vi "Open.vi"(8 "error in (no error)":errorcluster, 10 "App Refnum":refnum<vi>, 11 "LVUnit Test Case in":refnum<class "LVUnit Test Case.lvclass">) -> (0 "error out":errorcluster, 3 "LVUnit Test Case out":refnum<class "LVUnit Test Case.lvclass">)   [LabVIEW 2017, in "LVUnit Test Case.lvclass"]
doc: "Opens the document associated with the test case in the provided application context."
uses:
  LVUnit Test Case.lvclass
  C:/Users/pasca/Projects/Home/lvunit/Test Case/Test Case.lvclass
  Test Case/Test Case.lvclass/Test Case.ctl
  LVUnit Test Case.lvclass/LVUnit Test Case.ctl
  Test Case/Get Path.vi
  Get JSON Data.vi
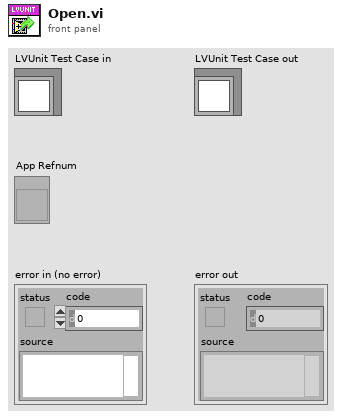
[diagram p1: front panel]
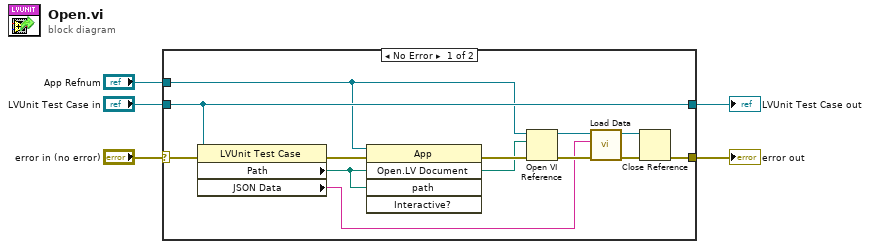
[diagram p0: block diagram]
diagram:
  n1 = case shown="No Error" "error in (no error)" {
    selector: "error in (no error)" -> [w17 w18]
    tunnel: "LVUnit Test Case in" -> [w16 w19]
    tunnel: [w8 w18] -> w3
    tunnel: [w16 w19] -> w2
    tunnel: "App Refnum" -> [w6 _]
    frame No Error {
      n2 = property class="LVUnit Test Case"(reference=w16, error in=w17) -> (error out=w11:errorcluster, "Path"=w9:path, "JSON Data"=w12:string)  [unwired: 1 out]
      n3 = invoke class="App" method="Open.LV Document"(reference=w6, error in=w11, "path"=w9) -> (error out=w10:errorcluster)  [unwired: 2 in, 4 out]
      n4 = Open VI Reference(application reference (local)=w6, vi path=w9, error in (no error)=w10) -> (vi reference=w13:refnum<vi>, error out=w15:errorcluster)  [unwired: 3 in]
      n5 = call "Load Data.vi"("error in (no error)"=w15, "JSON Data"=w12, "VI Reference"=w13) -> ("error out"=w14:errorcluster, "VI Refnum out"=w7:refnum<vi>)  [unwired: 7 in]
      n6 = Close Reference(reference=w7, error in (no error)=w14) -> (error out=w8:errorcluster)
    }
    frame Error {
    }
  }
  "error out" <- w3
  "LVUnit Test Case out" <- w2
